vi "Globals.vi"() -> ()   [LabVIEW 2024]
panel:
  out "First":bool
  out "A5":dbl
  out "A4":dbl
  out "A3":dbl
  out "VOUT-1.25":dbl
  out "Resistance Amplified":dbl
  out "Resistance A3":dbl
  in  "Res Duty Cycle":dbl
  out "Conductivity":dbl
  out "Step":dbl
  out "VREFs":dbl[](array[numeric])
  out "Stop":bool
  out "Auto":bool
  out "Target TC":dbl
  out "Target TH":dbl
  out "Elapsed Time":dbl
  out "Start Time":dbl
  in  "Data Array":string[][](array[string])=[["Time", "TH", "TC", "VOUT-1.25", "VREFs", "S", "A3", "A4", "A5", "R A3", "R Amplified"]]
  out "Voltage":dbl
  out "TC":dbl
  out "TH":dbl
  out "Seebeck Coefficient":dbl
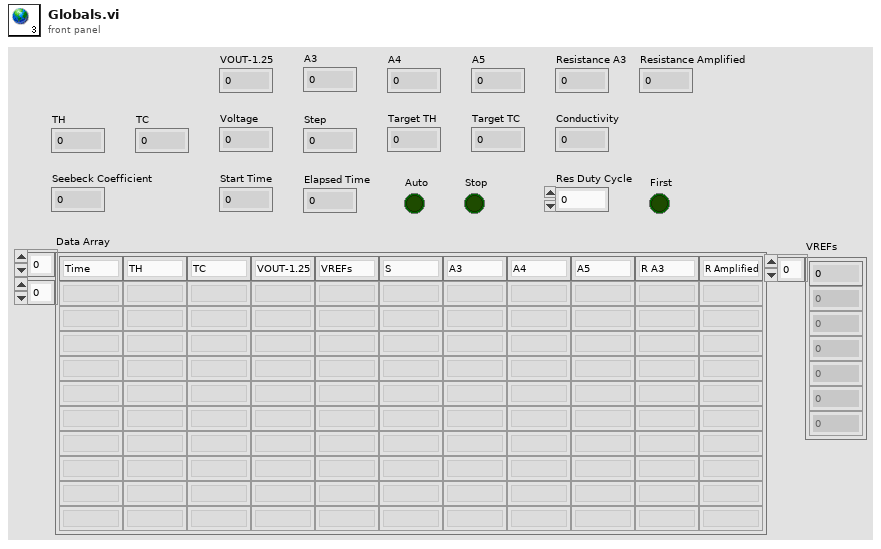
[diagram p1: front panel]
diagram:
